vi "Get Connections Impl.vi"(4 "pin type":T1, 6 "site":i32, 8 "error in":errorcluster, 9 "session factory":refnum<class "ISession Factory.lvclass">, 10 "pin or relay names":string[](array[string]), 11 "session reservation in":refnum<class "Session Reservation.lvclass">) -> (0 "error out":errorcluster, 2 "connections":T2[](array[typedef]), 3 "session reservation out":refnum<class "Session Reservation.lvclass">)   [LabVIEW 2021, in "NI Session Management V1 Client.lvlib" / "Session Reservation.lvclass"]
doc: "Validates if the <B> pin or relay names </B> reservation is successful and gets the connection information for the interested pins or pin groups."
uses:
  Session Reservation.lvclass
  Connection with Session.ctl
  Connection.ctl
  Sessions/Instrument/ISession Factory/ISession Factory.lvclass
  Pin Type.ctl
  Session Reservation.lvclass/Session Reservation.ctl
  Measurements/Helpers/Error Strings Global Internal.vi
  <vilib>/Utility/error.llb/Error Cluster From Error Code.vi
  Connection Map/Connection Map.lvclass
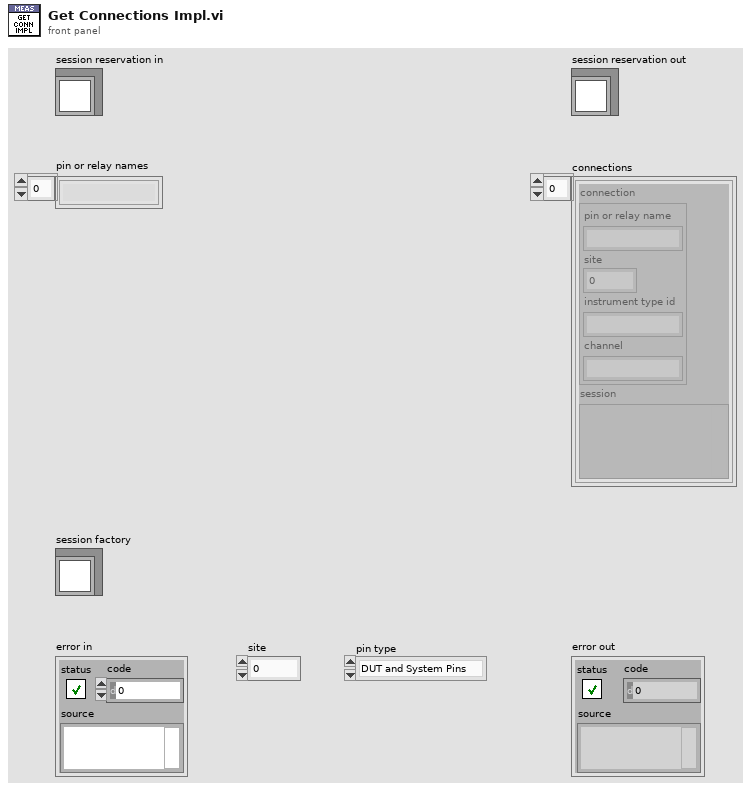
[diagram p1: front panel]
types:
  T1 = typedef "NI Session Management V1 Client.lvlib/Session Reservation.lvclass/Pin Type.ctl" = enum16{"DUT and System Pins", "System Pins"}
  T2 = typedef "NI Session Management V1 Client.lvlib/Session Reservation.lvclass/Connection with Session.ctl" = cluster{"connection":T3, "session":variant}
  T3 = typedef "NI Session Management V1 Client.lvlib/Session Reservation.lvclass/Connection.ctl" = cluster{"pin or relay name":string, "site":i32, "instrument type id":string, "channel":string}
  T4 = typedef "NI Session Management V1 Client.lvlib/Session Reservation.lvclass/Data.ctl" = cluster{"session and driver infos":T5[], "pin or relay names":string[], "connection map":refnum<class "Connection Map.lvclass">, "pin map context":T10, "reservation observer":refnum<class "IReservation Observer.lvclass">, "dvr valid":bool, "group mappings":T11}
  T5 = typedef "NI Session Management V1 Client.lvlib/Session Reservation.lvclass/Session and Driver Info.ctl" = cluster{"session info":T6, "session":variant, "session factory":refnum<class "ISession Factory.lvclass">, "initialize and close session behavior":T9}
  T6 = typedef "ni.measurementlink.sessionmanagement.v1.api.lvlib/ni_measurementlink_sessionmanagement_v1_SessionInformation.ctl" = cluster{"session":T7, "resource_name":string, "channel_list":string, "instrument_type_id":string, "session_exists":bool, "channel_mappings":T8[]}
  T7 = typedef "ni.measurementlink.sessionmanagement.v1.api.lvlib/nidevice_grpc_Session.ctl" = cluster{"name":string}
  T8 = typedef "ni.measurementlink.sessionmanagement.v1.api.lvlib/ni_measurementlink_sessionmanagement_v1_ChannelMapping.ctl" = cluster{"pin_or_relay_name":string, "site":i32, "channel":string, "multiplexer_resource_name":string, "multiplexer_route":string}
  T9 = typedef "NI Session Management Instrument.lvlib/ISession Factory.lvclass/Initialize and Close Session Behavior.ctl" = enum16{"Initialize and Close", "Attach and Detach", "Initialize and Detach", "Attach and Close"}
  T10 = typedef "ni.measurementlink.sessionmanagement.v1.api.lvlib/ni_measurementlink_PinMapContext.ctl" = cluster{"pin_map_id":string, "sites":i32[]}
  T11 = typedef "NI Session Management V1 Client.lvlib/Session Reservation.lvclass/Group Mapping.ctl" = map{string, string[]}
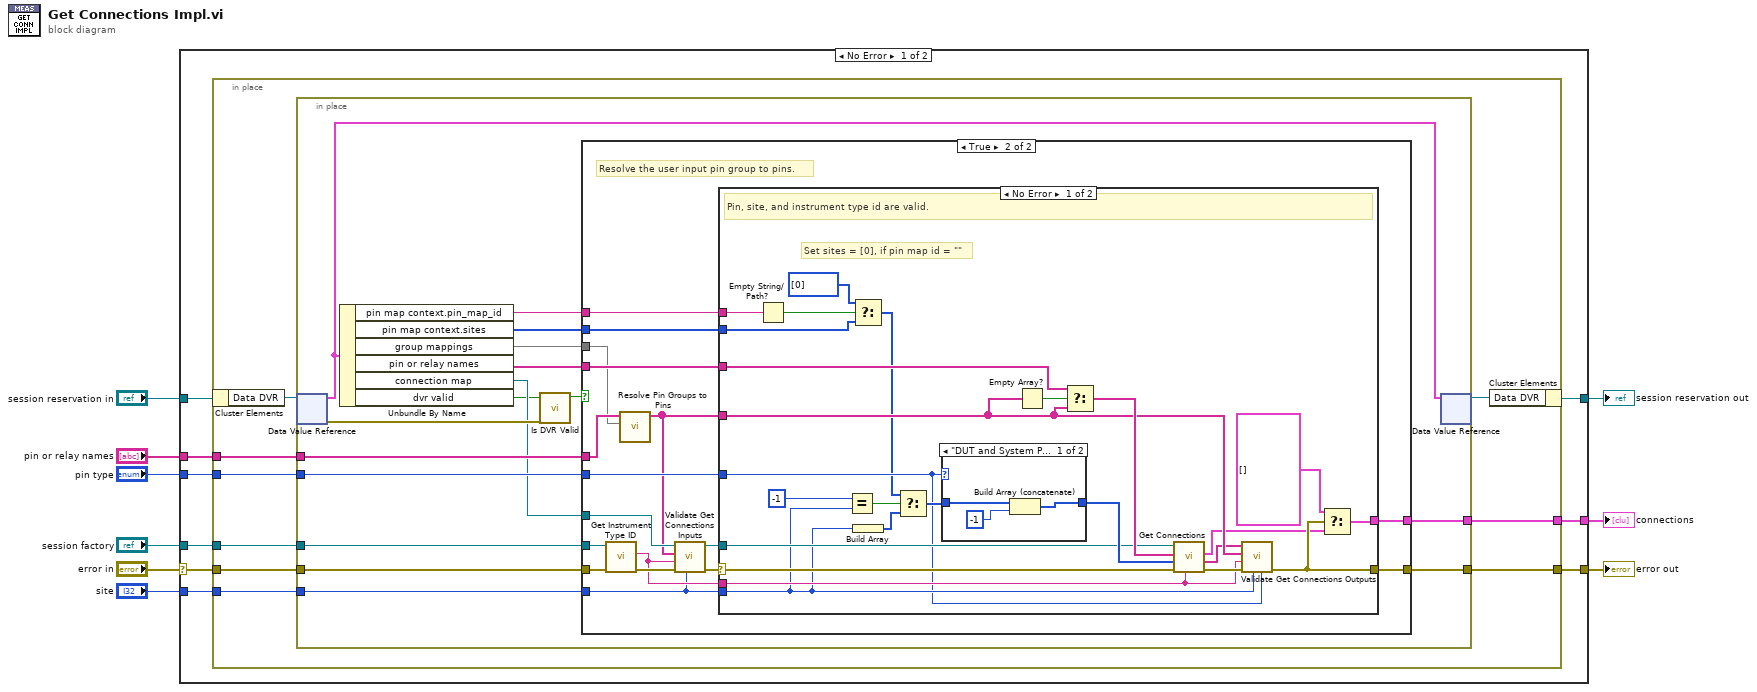
[diagram p0: block diagram]
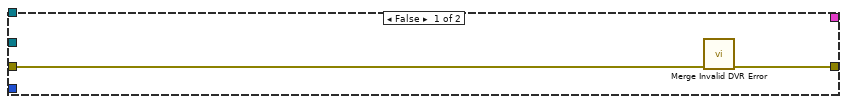
[diagram p2: hidden frame]
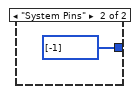
[diagram p3: hidden frame]
diagram:
  n1 = case shown="No Error" "error in" {
    selector: "error in" -> [w15 w94]
    tunnel: [w14 w94] -> w6
    tunnel: "session reservation in" -> [w12 w93]
    tunnel: "pin or relay names" -> [w18 _]
    tunnel: "site" -> [w17 _]
    tunnel: "session factory" -> [w16 _]
    tunnel: [w13 _] -> w4
    tunnel: [w11 w93] -> w2
    tunnel: "pin type" -> [w10 _]
    frame No Error {
      n2 = in-place {
        in-place-border: w18 -> [w27]
        in-place-border: w17 -> [w26]
        in-place-border: w16 -> [w25]
        in-place-border: w15 -> [w24]
        in-place-border: [w23] -> w14
        in-place-border: [w22] -> w13
        in-place-border: w10 -> [w19]
        n3 = in-place-cluster #1(w12) -> ("Data DVR"=w21:refnum<data-value>)
        n4 = in-place {
          in-place-border: w27 -> [w43]
          in-place-border: w26 -> [w42]
          in-place-border: w25 -> [w41]
          in-place-border: w24 -> [w40]
          in-place-border: [w39] -> w23
          in-place-border: [w38] -> w22
          in-place-border: w19 -> [w34]
          n5 = in-place-dvr #2(w21) -> (w35:T4, w30:errorcluster)
          n6 = Unbundle By Name(w35) -> ("pin map context.pin_map_id"=w31:string, "pin map context.sites"=w32:i32[], "group mappings"=w33:T11, "pin or relay names"=w37:string[], "connection map"=w29:refnum<class "Connection Map.lvclass">, "dvr valid"=w28:bool)
          n7 = call "Is DVR Valid.vi"("dvr error in"=w30, "dvr valid in"=w28) -> ("dvr valid out"=w36:bool)  [unwired: 9 in]
          n8 = case shown="True" w36 {
            tunnel: w43 -> [_ w50]
            tunnel: w42 -> [_ w53]
            tunnel: w41 -> [_ w62]
            tunnel: w40 -> [w45 w61]
            tunnel: [w44 w60] -> w39
            tunnel: [_ w51] -> w38
            tunnel: w37 -> [_ w59]
            tunnel: w34 -> [_ w58]
            tunnel: w29 -> [_ w52]
            tunnel: w33 -> [_ w48]
            tunnel: w32 -> [_ w46]
            tunnel: w31 -> [_ w47]
            frame False {
              n9 = call "Merge Invalid DVR Error.vi"("error in"=w45) -> ("error out"=w44:errorcluster)  [unwired: 10 in]
            }
            frame True {
              # "Resolve the user input pin group to pins."
              n10 = call-dynamic "Get Instrument Type ID.vi"("error in"=w61, "session factory in"=w62) -> ("error out"=w57:errorcluster, "instrument type id"=w56:string)  [unwired: 7 in, 1 out]
              n11 = call "Resolve Pin Groups to Pins.vi"("group mappings"=w48, "pin or group names"=w50) -> ("resolved pin or relay names"=w49:string[])  [unwired: 9 in]
              n12 = call "Validate Get Connections Inputs.vi"("site"=w53, "error in"=w57, "instrument type id"=w56, "pin or relay names"=w49, "connection map"=w52) -> ("error out"=w55:errorcluster, "connection map out"=w54:refnum<class "Connection Map.lvclass">)  [unwired: 5 in]
              n13 = case shown="No Error" w55 {
                selector: w55 -> [w79 w92]
                tunnel: [w71 w92] -> w60
                tunnel: w59 -> [w83 _]
                tunnel: w58 -> [w72 _]
                tunnel: w56 -> [w74 _]
                tunnel: w54 -> [w78 _]
                tunnel: w49 -> [w76 _]
                tunnel: w53 -> [w73 _]
                tunnel: [w68 _] -> w51
                tunnel: w47 -> [w63 _]
                tunnel: w46 -> [w64 _]
                frame No Error {
                  # "Set sites = [0], if pin map id = \"\""
                  # "Pin, site, and instrument type id are valid."
                  n14 = Empty String/Path?(string/path=w63) -> (empty?=w65:bool)
                  n15 = Equal?(x=-1, y=w73) -> (x = y?=w86:bool)
                  n16 = Select(t=i32[] [0] ("sites"), s=w65, f=w64) -> (s? t:f=w67:i32[])
                  n17 = Build Array(w73) -> (w87:i32[])
                  n18 = Select(t=w67, s=w86, f=w87) -> (s? t:f=w81:i32[])
                  n19 = case shown="\"DUT and System Pins\"" w72 {
                    tunnel: w81 -> [w89 _]
                    tunnel: [w88 i32[] [-1] ("sites")] -> w80
                    frame "DUT and System Pins" {
                      n20 = Build Array (concatenate)(w89, -1 ("x")) -> (w88:i32[])
                    }
                    frame "System Pins" {
                    }
                  }
                  n21 = Empty Array?(array=w76) -> (empty?=w82:bool)
                  n22 = Select(t=w83, s=w82, f=w76) -> (s? t:f=w84:string[])
                  n23 = call "Get Connections.vi"("instrument type id"=w74, "error in"=w79, "sites"=w80, "pin or relay names"=w84, "connection map in"=w78) -> ("error out"=w77:errorcluster, "pin or relay names found"=w75:string[], "connections"=w70:T2[])  [unwired: 3 in, 1 out]
                  n24 = call "Validate Get Connections Outputs.vi"("pin type"=w72, "site"=w73, "error in"=w77, "instrument type id"=w74, "pin or relay names"=w76, "pin or relay names found"=w75) -> ("error out"=w71:errorcluster)  [unwired: 5 in]
                  n25 = Select(t=T2[] [], s=w71, f=w70) -> (s? t:f=w68:T2[])
                }
                frame Error {
                  # "Pin, site, or instrument type not in connections map."
                }
              }
            }
          }
          n26 = in-place-dvr #2(w35) -> (w20:refnum<data-value>)  [unwired: 1 out]
        }
        n27 = in-place-cluster #1("Data DVR"=w20) -> (w11:refnum<class "Session Reservation.lvclass">)
      }
    }
    frame Error {
    }
  }
  "error out" <- w6
  "connections" <- w4
  "session reservation out" <- w2
